vi "Watchdog Add Interrupt Action.vi"(4 "error in (no error)":errorcluster, 6 "Occurrence RefNum":refnum<k4>, 7 "watchdogID in":u64 format="%.0x") -> (0 "error out":errorcluster, 3 "watchdogID out":u64 format="%.0x")   [LabVIEW 2025]
doc: "<p>Configures the <a href=\"nihelplauncher://docs/csh?context=lvrt_lvrtconcepts_rt_watchdog\">watchdog object</a> to trigger an occurrence when the watchdog timer expires. Use this VI in the configuration stage of the application, prior to the Watchdog Enable VI.</p>"
uses:
  niwd4c.dll
panel:
  out "actionParam":u64 format="%.0x"
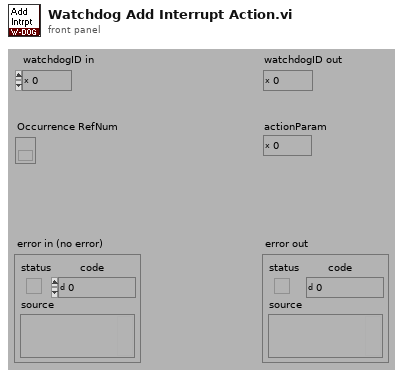
[diagram p1: front panel]
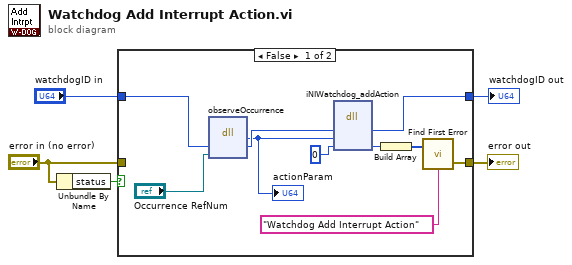
[diagram p0: block diagram]
diagram:
  n1 = Unbundle By Name("error in (no error)") -> ("status"=w5:bool)
  n2 = case shown="False" w5 {
    tunnel: [w11 w16] -> w1
    tunnel: [w14 w17] -> w2
    tunnel: "error in (no error)" -> [_ w17]
    tunnel: "watchdogID in" -> [w8 w16]
    frame False {
      n3 = dll-call lib="niwd4c.*" fn="observeOccurrence"("wd"=w8, "occurrence"="Occurrence RefNum") -> ("return type"=w6:u64, "wd"=w7:u64)  [unwired: 4 in, 2 out]
      "actionParam" <- w6
      n4 = dll-call lib="niwd4c.*" fn="iNIWatchdog_addAction" label="Add Action"("wd"=w7, "parameter"=w6, "status"=0) -> ("wd"=w11:u64, "status"=w12:i32)  [unwired: 5 in, 2 out]
      n5 = Build Array(w12) -> (w15:i32[])
      n6 = call <vilib>:"Find First Error.vi"("source messages"="Watchdog Add Interrupt Action", "error codes"=w15) -> ("error out"=w14:errorcluster)  [unwired: 2 in, 1 out]
    }
    frame True {
    }
  }
  "error out" <- w2
  "watchdogID out" <- w1
